vi "Get Policy Details.vi"(8 "error in (no error)":errorcluster, 10 "Name":string, 11 "IoT Session in":refnum<class "IoT Session.lvclass">) -> (0 "error out":errorcluster, 2 "Details":T1, 3 "IoT Session out":refnum<class "IoT Session.lvclass">)   [LabVIEW 2015, in "NI_AWS_IoT.lvlib" / "IoT Session.lvclass"]
uses:
  IoT Session.lvclass
  Policy.ctl
  Core/HTTP Request/Request Options.ctl
  Core/HTTP Request/Name Value Pair.ctl
  Core/HTTP Request/Region handling.ctl
  Core/HTTP Request/URL formatting.ctl
  Core/HTTP Request/HTTP Request.lvclass
  JSON Parsing/NI_JSON Parsing.lvlib
  NI_AWS_IoT.lvlib
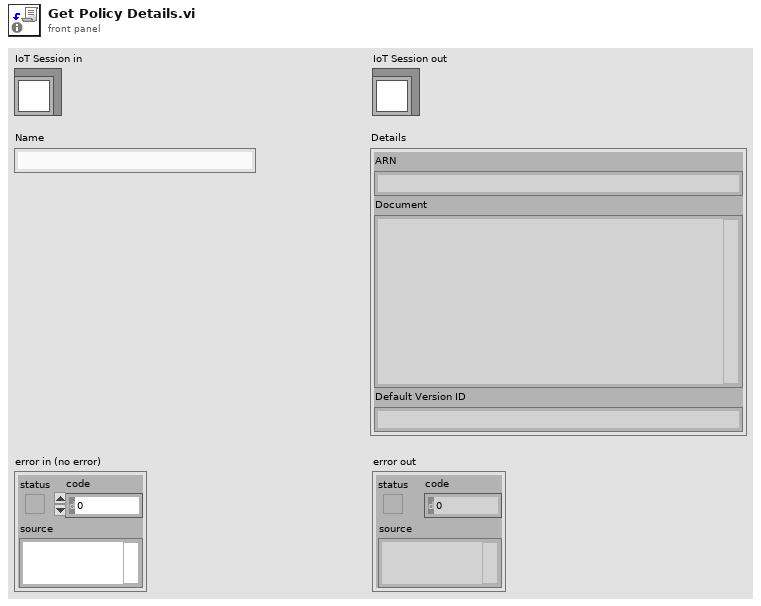
[diagram p1: front panel]
types:
  T1 = typedef "NI_AWS_IoT.lvlib/Policy.ctl" = cluster{"ARN":string, "Document":string, "Default Version ID":string}
  T2 = typedef "NI_AWS_Core.lvlib/HTTP Request.lvclass/Name Value Pair.ctl" = cluster{"name":string, "value":string}
  T3 = typedef "NI_AWS_Core.lvlib/HTTP Request.lvclass/Request Options.ctl" = cluster{"request headers":T2[], "request parameters":T2[], "request body":string, "region handling":T4, "URL formatting":T5}
  T4 = typedef "NI_AWS_Core.lvlib/HTTP Request.lvclass/Region handling.ctl" = enum16{"use region everywhere", "use region (authentication only)", "use region (URL only)", "ignore region everwhere"}
  T5 = typedef "NI_AWS_Core.lvlib/HTTP Request.lvclass/URL formatting.ctl" = enum16{"region-", "region."}
  T6 = typedef "NI_AWS_Core.lvlib/HTTP Request.lvclass/Response.ctl" = cluster{"Headers":string, "Body":string}
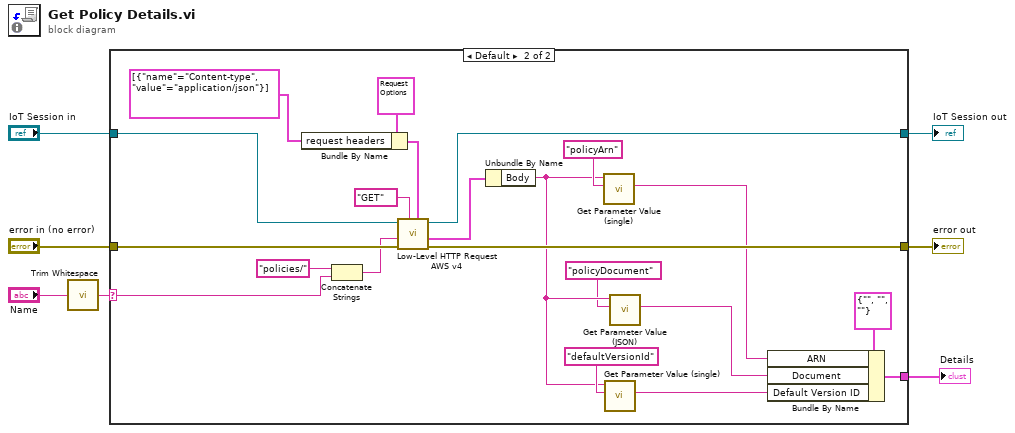
[diagram p0: block diagram]
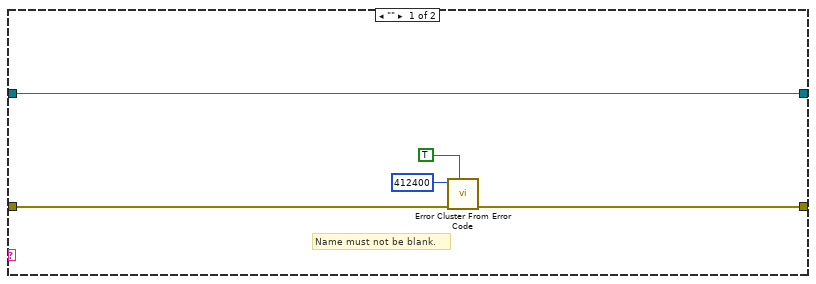
[diagram p2: hidden frame]
diagram:
  n1 = call <vilib>:"Trim Whitespace.vi"("string"="Name") -> ("trimmed string"=w1:string)  [unwired: 1 in]
  n2 = case shown="Default" w1 {
    selector: w1 -> [_ w21]
    tunnel: "error in (no error)" -> [w9 w33]
    tunnel: [w8 w32] -> w6
    tunnel: [w12 w31] -> w5
    tunnel: "IoT Session in" -> [w12 w30]
    tunnel: [_ w19] -> w2
    frame "" {
      # "Name must not be blank."
      n3 = call <vilib>:"Error Cluster From Error Code.vi"("show call chain? (False)"=TRUE, "error in (no error)"=w9, "error code (0)"=412400) -> ("error out"=w8:errorcluster)  [unwired: 6 in]
    }
    frame Default {
      n4 = Bundle By Name(cluster=T3 {"request headers"=[], "request parameters"=[], "request body"="", "region handling"=enum."use region everywhere", "URL formatting"=enum."region."} ("Request Options"), "request headers"=T2[] [{"name"="Content-type", "value"="application/json"}]) -> (w27:T3)
      n5 = Concatenate Strings("policies/" ("string"), w21) -> (w22:string)
      n6 = call "Low-Level HTTP Request AWS v4.vi"("Request Options"=w27, "HTTP-Verb"="GET", "error in (no error)"=w33, "URL Suffix"=w22, "AWS Core in"=w30) -> ("error out"=w32:errorcluster, "Response"=w25:T6, "AWS Core out"=w31:refnum<class "IoT Session.lvclass">)  [unwired: 3 in, 1 out]
      n7 = Unbundle By Name(w25) -> ("Body"=w15:string)
      n8 = call "Get Parameter Value (single).vi"("Parameter Name"="policyArn", "JSON"=w15) -> ("Parameter Value"=w18:string)  [unwired: 6 in, 3 out]
      n9 = call "Get Parameter Value (single).vi"("Parameter Name"="defaultVersionId", "JSON"=w15) -> ("Parameter Value"=w16:string)  [unwired: 6 in, 3 out]
      n10 = call "Get Parameter Value (JSON).vi"("Parameter Name"="policyDocument", "JSON"=w15) -> ("Parameter Value"=w13:string)  [unwired: 6 in, 3 out]
      n11 = Bundle By Name(cluster=T1 {"ARN"="", "Document"="", "Default Version ID"=""} ("Details"), "ARN"=w18, "Document"=w13, "Default Version ID"=w16) -> (w19:T1)
    }
  }
  "error out" <- w6
  "IoT Session out" <- w5
  "Details" <- w2
